vi "Write Writer Reference.vi"(8 "error in (no error)":errorcluster, 10 "BB Writer Refnum":T1 {"refnum" format="%.0x"}, 11 "CIF_Iceoryx_BB in":refnum<class "CIF_Iceoryx_BB.lvclass">) -> (0 "error out":errorcluster, 3 "CIF_Iceoryx_BB out":refnum<class "CIF_Iceoryx_BB.lvclass">)   [LabVIEW 2021, in "CIF_Iceoryx_BB.lvclass"]
uses:
  CIF_Iceoryx_BB.lvclass
  CIF_Iceoryx_BB.lvclass/CIF_Iceoryx_BB.ctl
  <vilib>/CIF Foundation/CIF Iceoryx/Refnum/Typedef/BB Writer Refnum.ctl
  <vilib>/CIF Foundation/CIF Iceoryx/Iceoryx.lvlib
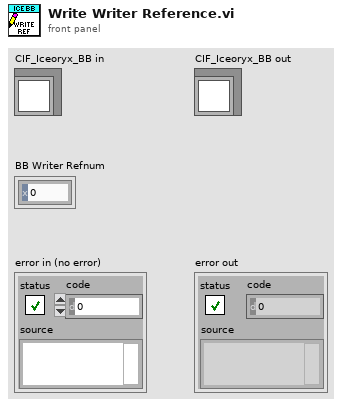
[diagram p1: front panel]
types:
  T1 = typedef "Iceoryx.lvlib/BB Writer Refnum.ctl" = cluster{"refnum":u64, "BB Writer":enum8{"bb_writer"}}
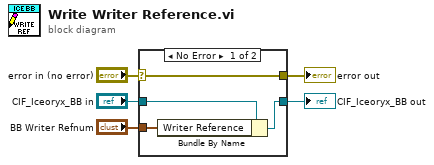
[diagram p0: block diagram]
diagram:
  n1 = case shown="No Error" "error in (no error)" {
    selector: "error in (no error)" -> [w9 w10]
    tunnel: [w9 w10] -> w4
    tunnel: [w7 w11] -> w2
    tunnel: "CIF_Iceoryx_BB in" -> [w8 w11]
    tunnel: "BB Writer Refnum" -> [w6 _]
    frame No Error {
      n2 = Bundle By Name(cluster=w8, "Writer Reference"=w6) -> (w7:refnum<class "CIF_Iceoryx_BB.lvclass">)
    }
    frame Error {
    }
  }
  "error out" <- w4
  "CIF_Iceoryx_BB out" <- w2
